vi "create default channels.vi"() -> (0 "error out":errorcluster, 1 "names":string[](array[string]), 2 "channels":refnum<class "TBM channel.lvclass">[](array[class]), 3 "module":refnum<class "alarms module configuration.lvclass">, 5 "instance identifier":string)   [LabVIEW 2013, in "alarms module tests.lvlib"]
uses:
  alarms module tests.lvlib
  <vilib>/NI/Tag Bus Module Framework/channel/TBM channel.lvclass
  module/configuration/alarms module configuration.lvclass
  module/configuration/compare type.ctl
  <vilib>/NI/Configuration Framework/serializable configuration/NISE_CEF_serializable configuration.lvclass
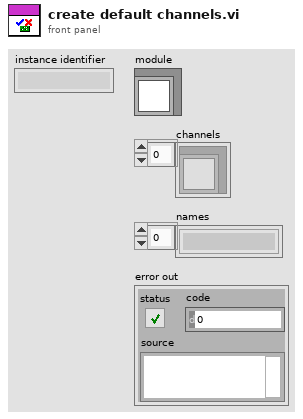
[diagram p1: front panel]
types:
  T1 = typedef "tag bus.lvlib/tag descriptor.lvclass/Data Type.ctl" = enum16{"Double", "Single", "I64", "I32", "I16", "I8", "U64", "U32", "U16", "U8", "Boolean", "String", "Array of Double", "Array of Single", "Array of I64", "Array of I32", "Array of I16", "Array of I8", "Array of U64", "Array of U32", "Array of U16", "Array of U8", "Array of Boolean", "Array of String"}
  T2 = typedef "alarms module configuration.lvclass/compare type.ctl" = enum16{">", "<", ">=", "<=", "="}
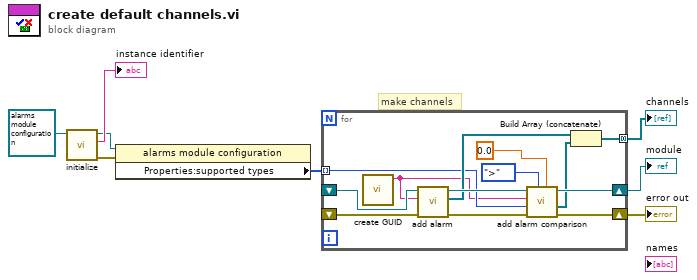
[diagram p0: block diagram]
diagram:
  # "make channels"
  n1 = call <vilib>:"initialize.vi"("configuration in"=refnum<class "alarms module configuration.lvclass"> refnum ("tag bus configurable plugin module configuration")) -> ("error out"=w7:errorcluster, "identifier"=→"instance identifier":string, "configuration out"=w6:refnum<class "alarms module configuration.lvclass">)  [unwired: 8 in]
  n2 = property class="alarms module configuration"(reference=w6, error in=w7) -> ("Properties:supported types"=w4:T1[])  [unwired: 2 out]
  n3 = for {
    tunnel: w4 -> [w12] mode=indexing
    shift-right: [w19] -> w2
    shift-left: _ -> [w20]
    tunnel: [w15] -> w3 mode=concatenating
    shift-right: [w14] -> w1
    shift-left: _ -> [w13]
    n4 = call <vilib>:"create GUID.vi"() -> ("uuid"=w11:string)  [unwired: 10 in, 1 out]
    n5 = call "add alarm.vi"("error in"=w13, "alarm name"=w11, "alarms module configuration in"=w20) -> ("error out"=w18:errorcluster, "created channels"=w17:refnum<class "TBM channel.lvclass">[], "alarms module configuration out"=w21:refnum<class "alarms module configuration.lvclass">)  [unwired: 6 in]
    n6 = call "add alarm comparison.vi"("Limit"=0.0, "comparison"=compare_type.">", "error in"=w18, "data type"=w12, "alarm name"=w11, "alarms module configuration in"=w21) -> ("error out"=w14:errorcluster, "created channels"=w16:refnum<class "TBM channel.lvclass">[], "alarms module configuration out"=w19:refnum<class "alarms module configuration.lvclass">)  [unwired: 2 in, 1 out]
    n7 = Build Array (concatenate)(w17, w16) -> (w15:refnum<class "TBM channel.lvclass">[])
  }
  "error out" <- w1
  "channels" <- w3
  "module" <- w2
